vi "Read Serial.vi"() -> ()   [LabVIEW 2014]
uses:
  <vilib>/Instr/_visa.llb/VISA Configure Serial Port (Instr).vi
panel:
  out "Waveform Chart":cluster{dbl, dbl}(graph)
  out "before substring":string
  out "after substring":string
  out "offset past match":i32
  in  "VISA resource name":refnum<visa-resource-name>
  out "element":string
  in  "baud rate (9600)":u32=9600
  in  "Stop Button":bool
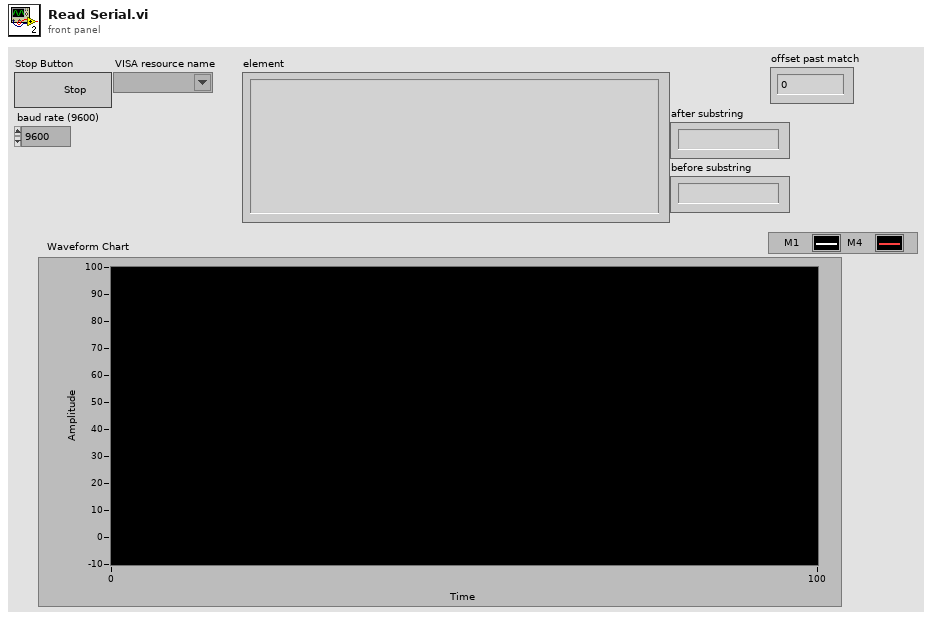
[diagram p1: front panel]
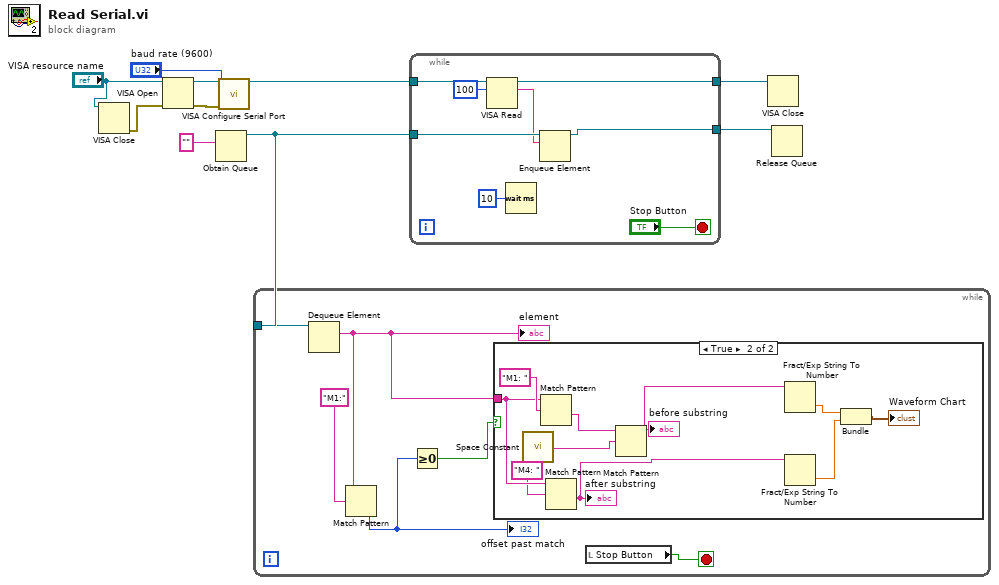
[diagram p0: block diagram]
diagram:
  n1 = VISA Close(VISA resource name="VISA resource name") -> (error out=w2:errorcluster)  [unwired: 1 in]
  n2 = VISA Open(error in (no error)=w2, VISA resource name="VISA resource name") -> (VISA resource name=w8:refnum<visa-resource-name>, error out=w7:errorcluster)  [unwired: 3 in]
  n3 = Obtain Queue(element data type="") -> (queue out=w10:refnum<queue>)  [unwired: 4 in, 2 out]
  n4 = call-poly "VISA Configure Serial Port"("VISA resource name"=w8, "baud rate (9600)"="baud rate (9600)", "error in (no error)"=w7) -> ("VISA resource name out"=w5:refnum<visa-resource-name>)  [unwired: 11 in, 1 out]
  n5 = while {
    tunnel: w10 -> [w16]
    stop <- w15 stop-if-true
    n6 = Dequeue Element(queue=w16) -> (element=w14:string)  [unwired: 2 in, 3 out]
    "element" <- w14
    n7 = Match Pattern(string=w14, regular expression="M1:" ("format string")) -> (offset past match=w12:i32)  [unwired: 1 in, 3 out]
    "offset past match" <- w12
    n8 = Greater Or Equal To 0?(x=w12) -> (x >= 0?=w11:bool)
    n9 = case shown="True" w11 {
      tunnel: w14 -> [_ w23]
      frame False {
      }
      frame True {
        n10 = call <vilib>:"Space Constant.vi"() -> ("String"=w24:string)
        n11 = Match Pattern(string=w23, regular expression="M1: " ("format string")) -> (after substring=w25:string)  [unwired: 1 in, 3 out]
        n12 = Match Pattern(string=w23, regular expression="M4: " ("format string")) -> (after substring=w20:string)  [unwired: 1 in, 3 out]
        "after substring" <- w20
        n13 = Match Pattern(string=w25, regular expression=w24) -> (before substring=w21:string)  [unwired: 1 in, 3 out]
        "before substring" <- w21
        n14 = Fract/Exp String To Number(string=w21) -> (number=w19:dbl)  [unwired: 3 in, 1 out]
        n15 = Fract/Exp String To Number(string=w20) -> (number=w18:dbl)  [unwired: 3 in, 1 out]
        n16 = Bundle(w19, w18) -> (→"Waveform Chart":cluster{dbl, dbl})  [unwired: 1 in]
      }
    }
    n17 = local read "Stop Button"() -> (w15:bool)
  }
  n18 = while {
    tunnel: w10 -> [w34]
    tunnel: w5 -> [w32]
    tunnel: [w29] -> w4
    tunnel: [w28] -> w3
    stop <- "Stop Button" stop-if-true
    n19 = VISA Read(VISA resource name=w32, byte count=u32 100) -> (VISA resource name out=w29:refnum<visa-resource-name>, read buffer=w31:string)  [unwired: 1 in, 2 out]
    n20 = Wait (ms)(milliseconds to wait=u32 10) -> ()  [unwired: 1 out]
    n21 = Enqueue Element(queue=w34, element=w31) -> (queue out=w28:refnum<queue>)  [unwired: 2 in, 2 out]
  }
  n22 = VISA Close(VISA resource name=w4) -> ()  [unwired: 1 in, 1 out]
  n23 = Release Queue(queue=w3) -> ()  [unwired: 2 in, 3 out]
